vi "AddDesignPatterns.vi"(0 "ClassWriterNative":refnum<class "ClassWriterNative.lvclass">, 1 "ClassItemRefIn":refnum<vi>, 2 "DesignPatterns":string[](array[string]), 5 "error in (no error)":errorcluster) -> (14 "ClassWriterNative":refnum<class "ClassWriterNative.lvclass">, 15 "ClassItemRefOut":refnum<vi>, 17 "Cancelled":bool, 19 "error out":errorcluster)   [LabVIEW 2020, in "ClassWriterNative.lvclass"]
uses:
  ClassWriterNative.lvclass
  Provider_BaseClassInterface/DesignPatternsData.ctl
  Common/LvClass_class/GDSLvClass_PlugIn.ctl
  Common/LvClass_class/GDSLvClass_PlugInTypes.ctl
  Provider_BaseClassInterface/BaseProvider_SubVIs/BaseProvider_DesignPatternsActions.ctl
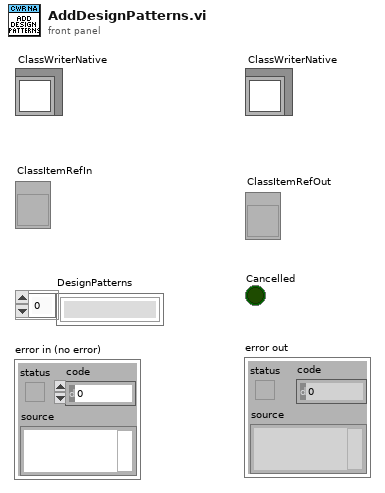
[diagram p1: front panel]
types:
  T1 = typedef "DesignPatternsData.ctl" = cluster{"Type":string, "Patterns":cluster{"ID":string, "Path":path, "Name":string, "Desc":string, "Version":string, "DependenciesID":string[], "OnlyOne":bool}[]}
  T2 = cluster{"Cancel":bool, "ClassProviderName":string, "ClassTemplateUsed":string, "DesignPatterns":T1[], "DataOut":variant, "PlugInVI":path, "DesignPatternID":string, "DesignPatternType":string, "PlugInIDs":string[], "DesignPatternVer":string, "DPIDs":string[], "DpToAdd":cluster{"ID":string, "Path":path, "Name":string, "Desc":string, "Version":string, "DependenciesID":string[], "OnlyOne":bool}[]}
  T3 = cluster{"ID":string, "Path":path, "Name":string, "Desc":string, "Version":string, "DependenciesID":string[], "OnlyOne":bool}[]
  T4 = typedef "GDSLvClass_PlugIn.ctl" = cluster{"Type":T5, "ID":string, "Version":string, "Path":path, "Name":string, "Data":variant}
  T5 = typedef "GDSLvClass_PlugInTypes.ctl" = enum16{"DesignPattern", "MethodTypes"}
  T6 = typedef "BaseProvider_DesignPatternsActions.ctl" = enum16{"AddPatternDialog", "GeneratePattern", "RemovePattern", "CreatePatternMethod", "UpdatePattern"}
  T7 = typedef "GDSLvCLass_ClassSettingsType.ctl" = cluster{"ClassProviderName":string, "ClassTemplateUsed":string, "ClassTemplateVersion":string, "ClassDescription":string, "PlugIns":T4[], "ConnectorPanePattern":string}
  T8 = cluster{"ID":string, "Path":path, "Name":string, "Desc":string, "Version":string, "DependenciesID":string[], "OnlyOne":bool}
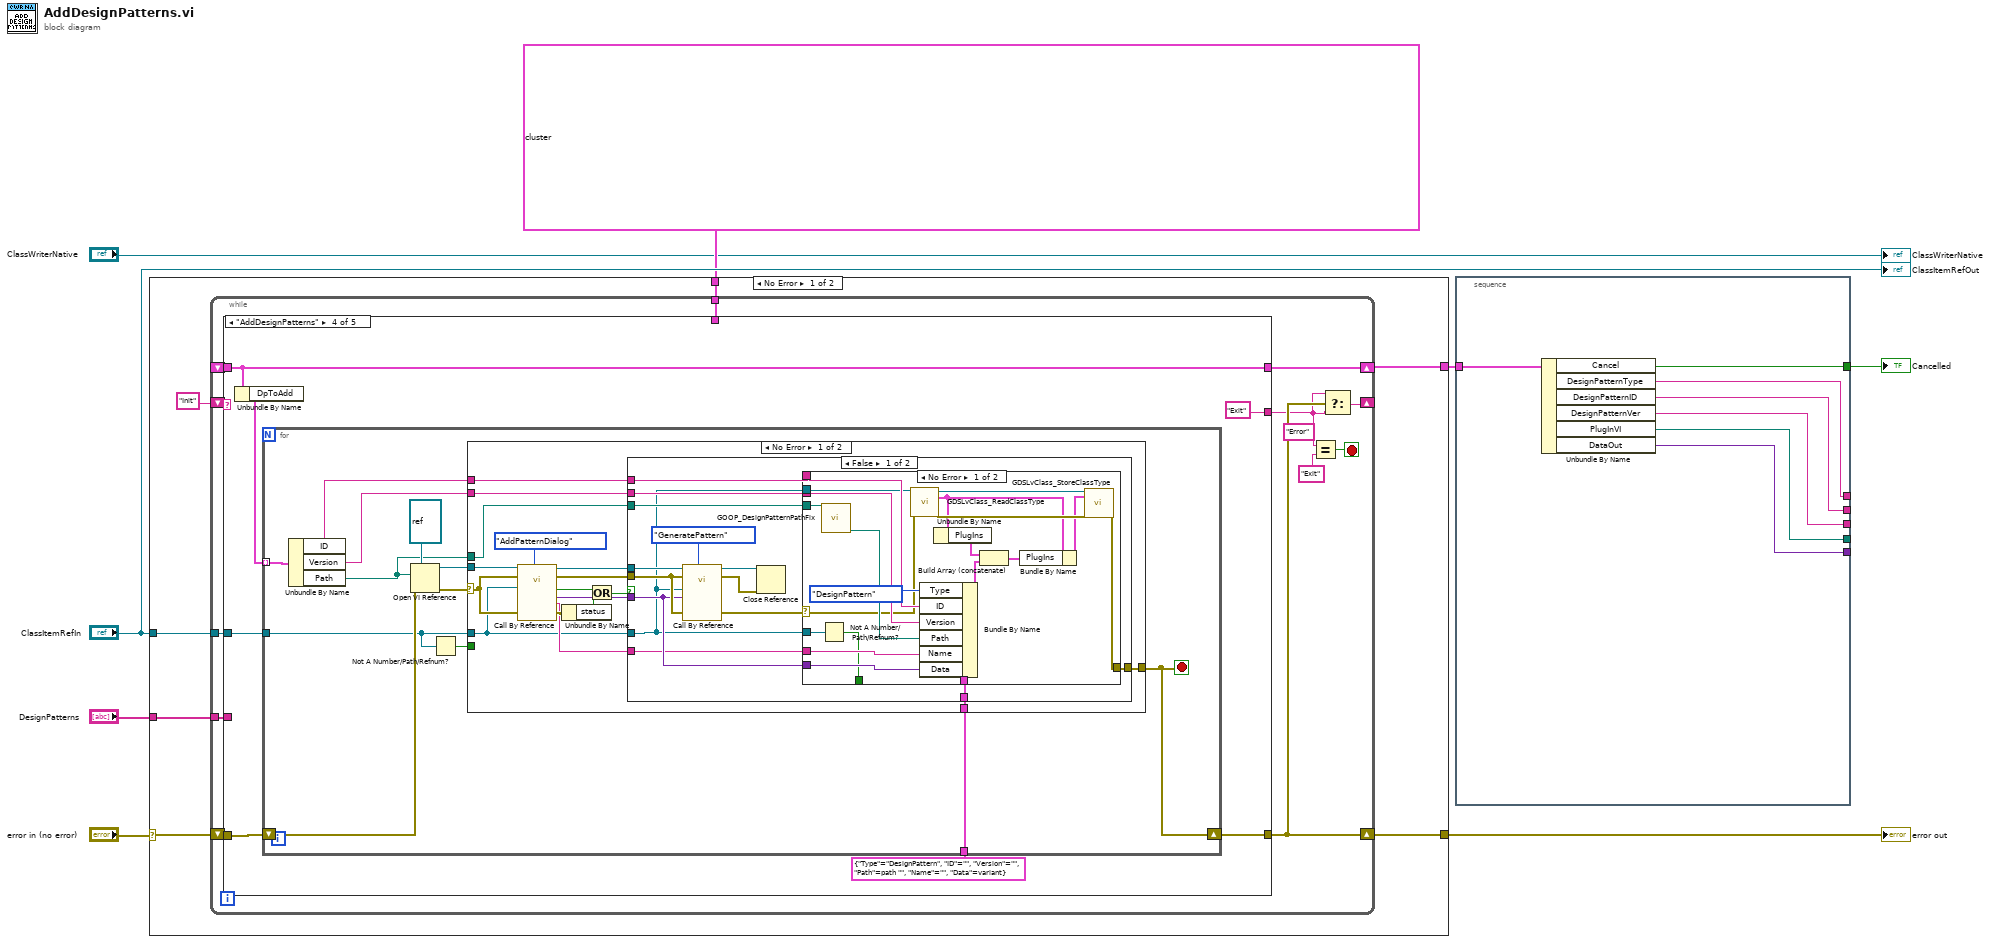
[diagram p0: block diagram]
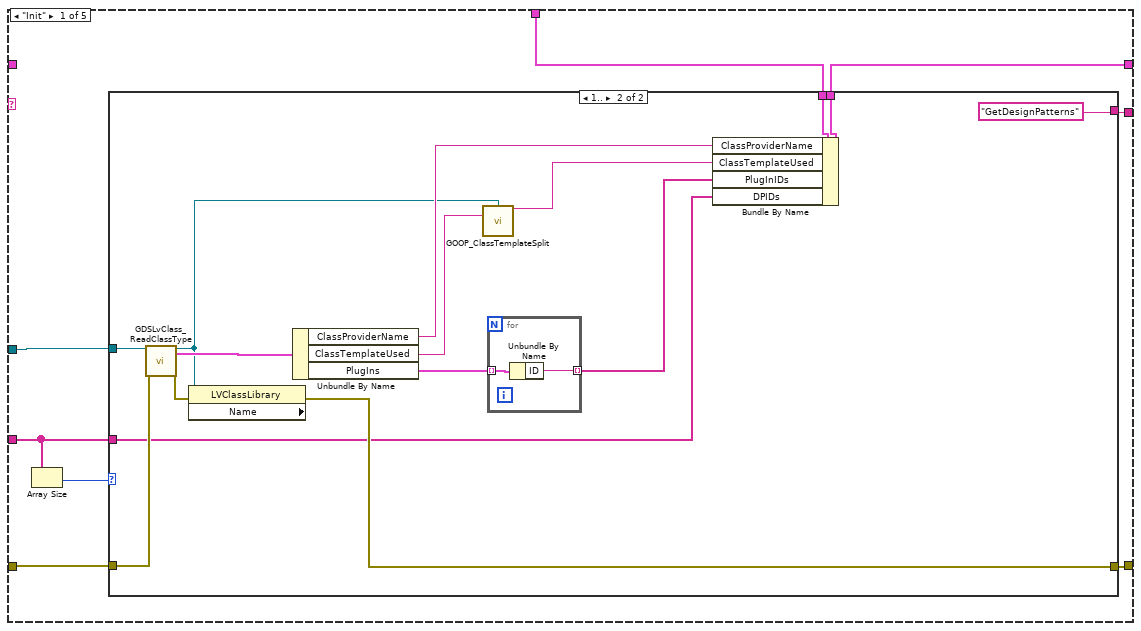
[diagram p2: hidden frame]
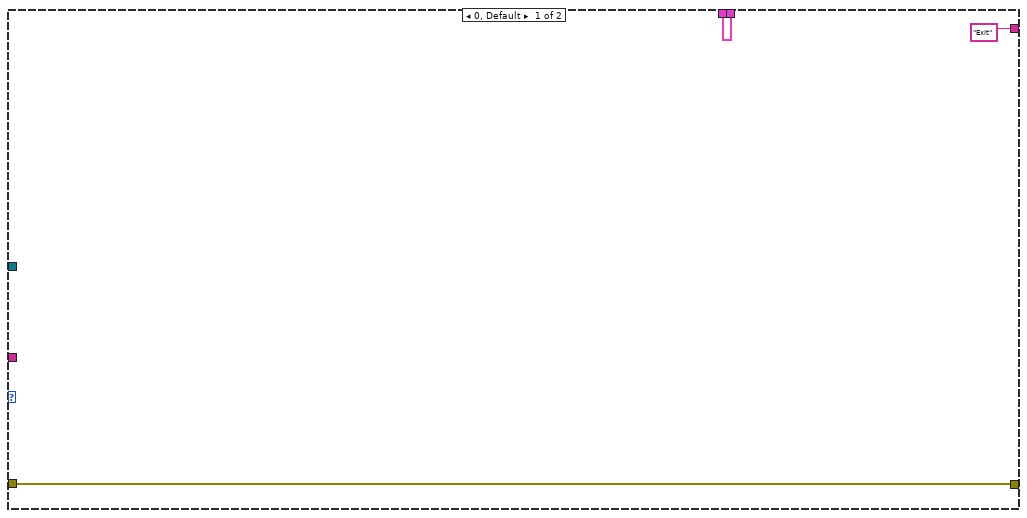
[diagram p3: hidden frame]
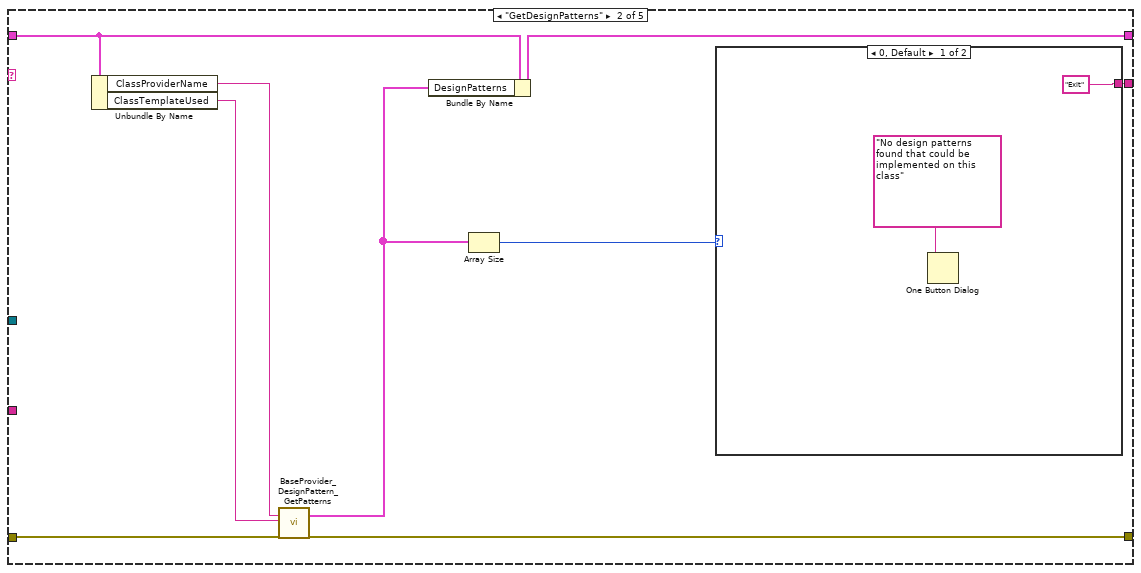
[diagram p4: hidden frame]
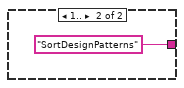
[diagram p5: hidden frame]
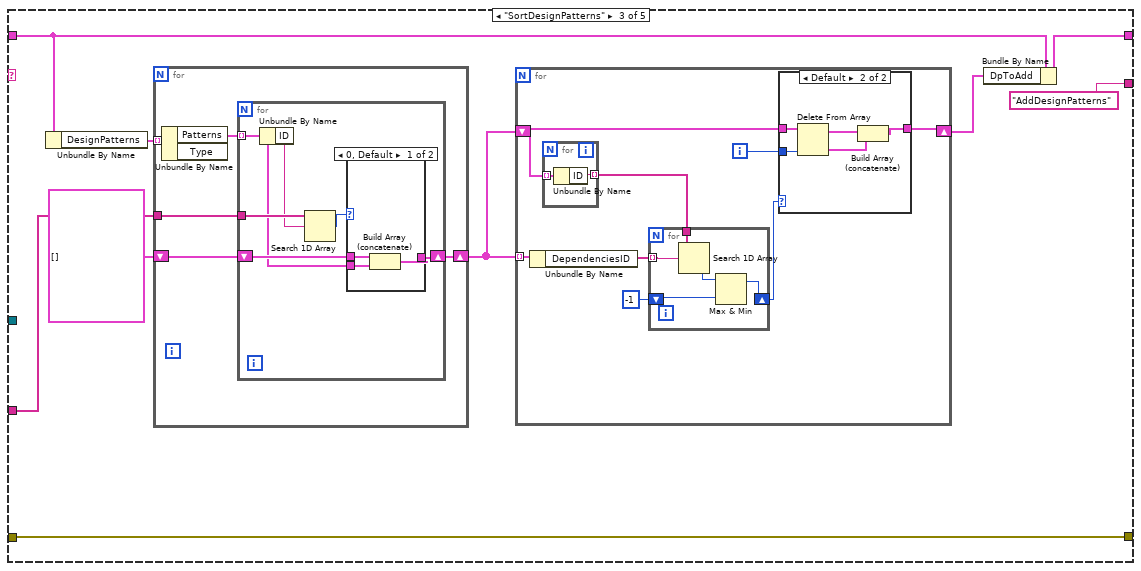
[diagram p6: hidden frame]
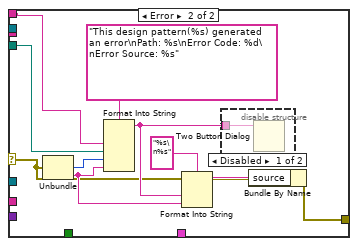
[diagram p9: hidden frame]
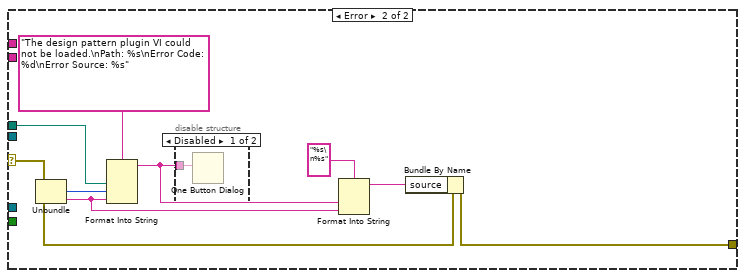
[diagram p12: hidden frame]
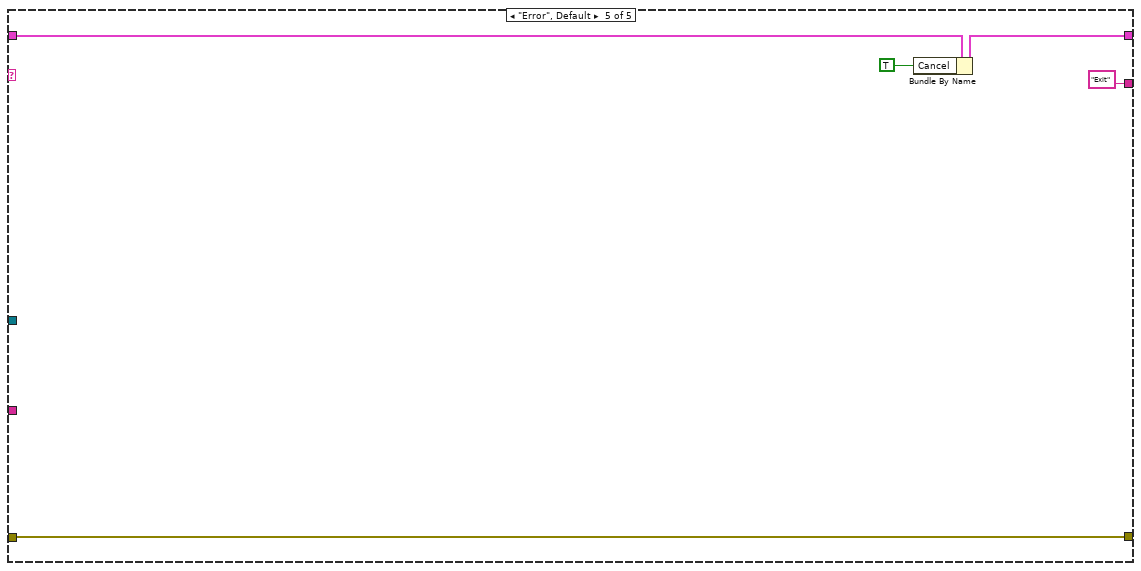
[diagram p14: hidden frame]
diagram:
  n1 = case shown="No Error" "error in (no error)" {
    selector: "error in (no error)" -> [w9 w211]
    tunnel: [w15 w211] -> w5
    tunnel: T2 {"Cancel"=FALSE, "ClassProviderName"="", "ClassTemplateUsed"="", "DesignPatterns"=[], "DataOut"=variant, "PlugInVI"=path "", "DesignPatternID"="", "DesignPatternType"="", "PlugInIDs"=[], "DesignPatternVer"="", "DPIDs"=[], "DpToAdd"=[]} ("output cluster") -> [w13 _]
    tunnel: "ClassItemRefIn" -> [w12 _]
    tunnel: [w11 _] -> w7
    tunnel: "DesignPatterns" -> [w10 _]
    frame No Error {
      n2 = while {
        shift-right: [w22] -> w15
        shift-left: w9 -> [w28]
        shift-right: [w21] -> _
        shift-left: "Init" -> [w25]
        shift-right: [w26] -> w11
        shift-left: _ -> [w27]
        tunnel: w13 -> [w18]
        tunnel: w12 -> [w17]
        tunnel: w10 -> [w16]
        stop <- w23 stop-if-true
        n3 = case shown="\"AddDesignPatterns\"" w25 {
          tunnel: w27 -> [_ w58 w72 w117 w208]
          tunnel: [w31 w57 w71 w117 w207] -> w26
          tunnel: w28 -> [w34 w63 w75 w119 w209]
          tunnel: [w33 w60 w75 w115 w209] -> w22
          tunnel: [w36 w65 "AddDesignPatterns" "Exit" "Exit"] -> w20
          tunnel: w18 -> [w32 _ _ _ _]
          tunnel: w17 -> [w35 _ _ w118 _]
          tunnel: w16 -> [w30 _ w74 _ _]
          frame "Init" {
            n4 = Array Size(array=w30) -> (size(s)=w29:i32)
            n5 = case shown="1.." w29 {
              tunnel: ["Exit" "GetDesignPatterns"] -> w36
              tunnel: w35 -> [_ w53]
              tunnel: w34 -> [w37 w52]
              tunnel: [w37 w49] -> w33
              tunnel: w32 -> [w39 w47]
              tunnel: [w39 w46] -> w31
              tunnel: w30 -> [_ w43]
              frame 0, Default {
              }
              frame 1.. {
                n6 = call "GDSLvClass_ReadClassType.vi"("Class Refnum In"=w53, "error in (no error)"=w52) -> ("Class Refnum Out"=w40:refnum<vi>, "ClassSettings"=w51:T7, "error out"=w50:errorcluster)  [unwired: 15 in]
                n7 = property class="LVClassLibrary" props=["Name"](reference=w40, error in=w50) -> (error out=w49:errorcluster)  [unwired: 2 out]
                n8 = Unbundle By Name(w51) -> ("ClassProviderName"=w48:string, "ClassTemplateUsed"=w42:string, "PlugIns"=w45:T4[])
                n9 = call "GOOP_ClassTemplateSplit.vi"("ClassItemRefIn"=w40, "FullClassTemplate"=w42) -> ("StandardTemplate"=w41:string)  [unwired: 12 in, 1 out]
                n10 = for {
                  tunnel: w45 -> [w56] mode=indexing
                  tunnel: [w55] -> w44 mode=indexing
                  n11 = Unbundle By Name(w56) -> ("ID"=w55:string)
                }
                n12 = Bundle By Name(cluster=w47, "ClassProviderName"=w48, "ClassTemplateUsed"=w41, "PlugInIDs"=w44, "DPIDs"=w43) -> (w46:T2)
              }
            }
          }
          frame "GetDesignPatterns" {
            n13 = Unbundle By Name(w58) -> ("ClassProviderName"=w62:string, "ClassTemplateUsed"=w61:string)
            n14 = call "BaseProvider_DesignPattern_GetPatterns.vi"("FilterOnProviders(Ignored If Empty)"=w62, "FilterOnTemplate(Ignored If Empty)"=w61, "error in (no error)"=w63) -> ("DesignPatterns"=w59:T1[], "error out"=w60:errorcluster)  [unwired: 15 in]
            n15 = Bundle By Name(cluster=w58, "DesignPatterns"=w59) -> (w57:T2)
            n16 = Array Size(array=w59) -> (size(s)=w64:i32)
            n17 = case shown="0, Default" w64 {
              tunnel: ["Exit" "SortDesignPatterns"] -> w65
              frame 0, Default {
                n18 = One Button Dialog(message="No design patterns found that could be implemented on this class" ("format string")) -> ()  [unwired: 1 in, 1 out]
              }
              frame 1.. {
              }
            }
          }
          frame "SortDesignPatterns" {
            n19 = Unbundle By Name(w72) -> ("DesignPatterns"=w76:T1[])
            n20 = for {
              tunnel: w76 -> [w103] mode=indexing
              tunnel: w74 -> [w101]
              shift-right: [w99] -> w73
              shift-left: T3 [] -> [w100]
              n21 = Unbundle By Name(w103) -> ("Patterns"=w102:T3)  [unwired: 1 out]
              n22 = for {
                tunnel: w102 -> [w104] mode=indexing
                tunnel: w101 -> [w109]
                shift-right: [w105] -> w99
                shift-left: w100 -> [w106]
                n23 = Unbundle By Name(w104) -> ("ID"=w108:string)
                n24 = Search 1D Array(1D array=w109, element=w108) -> (index of element=w107:i32)  [unwired: 1 in]
                n25 = case shown="0, Default" w107 {
                  tunnel: w106 -> [w112 w113]
                  tunnel: [w111 w113] -> w105
                  tunnel: w104 -> [w110 _]
                  frame 0, Default {
                    n26 = Build Array (concatenate)(w112, w110) -> (w111:T3)
                  }
                  frame -1 {
                  }
                }
              }
            }
            n27 = for {
              tunnel: w73 -> [w85] mode=indexing
              shift-right: [w79] -> w70
              shift-left: w73 -> [w81]
              i -> [w78]
              n28 = Unbundle By Name(w85) -> ("DependenciesID"=w84:string[])
              n29 = for {
                tunnel: w81 -> [w98] mode=indexing
                tunnel: [w97] -> w83 mode=indexing
                n30 = Unbundle By Name(w98) -> ("ID"=w97:string)
              }
              n31 = for {
                tunnel: w84 -> [w96] mode=indexing
                tunnel: w83 -> [w95]
                shift-right: [w92] -> w80
                shift-left: -1 -> [w93]
                n32 = Search 1D Array(1D array=w95, element=w96) -> (index of element=w94:i32)  [unwired: 1 in]
                n33 = Max & Min(x=w94, y=w93) -> (max(x,y)=w92:i32)  [unwired: 1 out]
              }
              n34 = case shown="Default" w80 {
                tunnel: w81 -> [w86 w91]
                tunnel: [w86 w87] -> w79
                tunnel: w78 -> [_ w90]
                frame -1 {
                }
                frame Default {
                  n35 = Delete From Array(array=w91, index=w90) -> (deleted portion=w88:T8, array with subset deleted=w89:T3)  [unwired: 1 in]
                  n36 = Build Array (concatenate)(w89, w88) -> (w87:T3)
                }
              }
            }
            n37 = Bundle By Name(cluster=w72, "DpToAdd"=w70) -> (w71:T2)
          }
          frame "AddDesignPatterns" {
            n38 = Unbundle By Name(w117) -> ("DpToAdd"=w120:T3)
            n39 = for {
              tunnel: w120 -> [w128] mode=indexing
              shift-right: [w121] -> w115
              shift-left: w119 -> [w127]
              tunnel: w118 -> [w123]
              tunnel: T4 {"Type"=enum."DesignPattern", "ID"="", "Version"="", "Path"=path "", "Name"="", "Data"=variant} ("PlugIn") -> [w126]
              stop <- w121 stop-if-true
              n40 = Unbundle By Name(w128) -> ("ID"=w125:string, "Version"=w124:string, "Path"=w129:path)
              n41 = Open VI Reference(type specifier VI Refnum (for type only)=refnum<vi> refnum, vi path=w129, error in (no error)=w127) -> (vi reference=w131:refnum<vi>, error out=w130:errorcluster)  [unwired: 3 in]
              n42 = Not A Number/Path/Refnum?(number/path/refnum=w123) -> (NaN/Path/Refnum?=w122:bool)
              n43 = case shown="No Error" w130 {
                selector: w130 -> [w141 w201]
                tunnel: w131 -> [w149 _]
                tunnel: w129 -> [w136 w202]
                tunnel: w123 -> [w134 _]
                tunnel: w126 -> [w139 _]
                tunnel: w125 -> [w138 _]
                tunnel: w124 -> [w137 _]
                tunnel: w122 -> [_ _]
                tunnel: [w133 w196] -> w121
                frame No Error {
                  n44 = call-by-ref "?"(reference=w149, error in=w141, "Action"=BaseProvider_DesignPatternsActions."AddPatternDialog", 8:"error in (no error)"=w141, "ClassRefToActOn"=w134) -> (reference out=w143:refnum<vi>, error out=w142:errorcluster, 0:"error out"=w148:errorcluster, "Name"=w135:string, "DataOut"=w140:variant, "Cancelled"=w147:bool)  [unwired: 5 in]
                  n45 = Unbundle By Name(w148) -> ("status"=w145:bool)
                  n46 = Or(x=w147, y=w145) -> (x .or. y?=w144:bool)
                  n47 = case shown="False" w144 {
                    tunnel: w143 -> [w163 _]
                    tunnel: w134 -> [w151 _]
                    tunnel: w142 -> [w161 w195]
                    tunnel: w140 -> [w156 _]
                    tunnel: w139 -> [w157 _]
                    tunnel: w138 -> [w155 _]
                    tunnel: w137 -> [w154 _]
                    tunnel: w136 -> [w153 _]
                    tunnel: w135 -> [w152 _]
                    tunnel: [w150 w195] -> w133
                    frame False {
                      n48 = call-by-ref "?"(reference=w163, error in=w161, "Action"=BaseProvider_DesignPatternsActions."GeneratePattern", 8:"error in (no error)"=w161, "DataIn"=w156, "ClassRefToActOn"=w151) -> (reference out=w160:refnum<vi>, error out=w159:errorcluster, 0:"error out"=w158:errorcluster)  [unwired: 4 in, 3 out]
                      n49 = Close Reference(reference=w160, error in (no error)=w159) -> ()  [unwired: 1 out]
                      n50 = case shown="No Error" w158 {
                        selector: w158 -> [w164 w185]
                        tunnel: w157 -> [w175 _]
                        tunnel: w156 -> [w174 _]
                        tunnel: w155 -> [w173 w191]
                        tunnel: w154 -> [w172 _]
                        tunnel: w153 -> [w167 w190]
                        tunnel: w151 -> [w171 _]
                        tunnel: w152 -> [w170 _]
                        tunnel: w151 -> [w169 _]
                        tunnel: [w168 _] -> _
                        tunnel: [w165 w184] -> w150
                        frame No Error {
                          n51 = Not A Number/Path/Refnum?(number/path/refnum=w169) -> (NaN/Path/Refnum?=w168:bool)
                          n52 = call "GOOP_DesignPatternPathFix.vi"("ViPathIn"=w167) -> ("RelativeVIPathOut(ToStoreInLvClass)"=w166:path)  [unwired: 6 in, 4 out]
                          n53 = call "GDSLvClass_ReadClassType.vi"("Class Refnum In"=w171, "error in (no error)"=w164) -> ("Class Refnum Out"=w183:refnum<vi>, "ClassSettings"=w180:T7, "error out"=w182:errorcluster)  [unwired: 15 in]
                          n54 = Bundle By Name(cluster=w175, "Type"=GDSLvClass_PlugInTypes."DesignPattern", "ID"=w173, "Version"=w172, "Path"=w166, "Name"=w170, "Data"=w174) -> (w177:T4)
                          n55 = Unbundle By Name(w180) -> ("PlugIns"=w179:T4[])
                          n56 = Build Array (concatenate)(w179, w177) -> (w178:T4[])
                          n57 = Bundle By Name(cluster=w180, "PlugIns"=w178) -> (w181:T7)
                          n58 = call "GDSLvClass_StoreClassType.vi"("Class Refnum In"=w183, "ClassSettings"=w181, "error in (no error)"=w182) -> ("error out"=w165:errorcluster)  [unwired: 15 in, 1 out]
                        }
                        frame Error {
                          n59 = Unbundle(w185) -> ("code"=w192:i32, "source"=w186:string)  [unwired: 1 out]
                          n60 = Format Into String(format string="This design pattern(%s) generated an error\nPath: %s\nError Code: %d\nError Source: %s" ("message"), w191, w190, w192, w186) -> (resulting string=w187:string)  [unwired: 2 in, 1 out]
                          n61 = Format Into String(format string="%s\n%s", w187, w186) -> (resulting string=w188:string)  [unwired: 2 in, 1 out]
                          n62 = disable-structure shown="Disabled" {
                            disable-tunnel: w187 -> [w194 _]
                            frame Disabled {
                              n63 = Two Button Dialog(message=w194) -> ()  [unwired: 2 in, 1 out]
                            }
                            frame Enabled {
                            }
                          }
                          n64 = Bundle By Name(cluster=w185, "source"=w188) -> (w184:errorcluster)
                        }
                      }
                    }
                    frame True {
                    }
                  }
                }
                frame Error {
                  n65 = Unbundle(w201) -> ("code"=w203:i32, "source"=w198:string)  [unwired: 1 out]
                  n66 = Format Into String(format string="The design pattern plugin VI could not be loaded.\nPath: %s\nError Code: %d\nError Source: %s" ("message"), w202, w203, w198) -> (resulting string=w199:string)  [unwired: 2 in, 1 out]
                  n67 = disable-structure shown="Disabled" {
                    disable-tunnel: w199 -> [w205 _]
                    frame Disabled {
                      n68 = One Button Dialog(message=w205) -> ()  [unwired: 1 in, 1 out]
                    }
                    frame Enabled {
                    }
                  }
                  n69 = Format Into String(format string="%s\n%s", w199, w198) -> (resulting string=w197:string)  [unwired: 2 in, 1 out]
                  n70 = Bundle By Name(cluster=w201, "source"=w197) -> (w196:errorcluster)
                }
              }
            }
          }
          frame "Error", Default {
            n71 = Bundle By Name(cluster=w208, "Cancel"=TRUE) -> (w207:T2)
          }
        }
        n72 = Equal?(x=w20, y="Exit") -> (x = y?=w23:bool)
        n73 = Select(t="Error", s=w22, f=w20) -> (s? t:f=w21:string)
      }
    }
    frame Error {
    }
  }
  "error out" <- w5
  n74 = stacked-sequence {
    tunnel: w7 -> [w218]
    tunnel: [w217] -> w6
    tunnel: [w216] -> _
    tunnel: [w215] -> _
    tunnel: [w214] -> _
    tunnel: [w213] -> _
    tunnel: [w212] -> _
    frame #0 {
      n75 = Unbundle By Name(w218) -> ("Cancel"=w217:bool, "DesignPatternType"=w213:string, "DesignPatternID"=w214:string, "DesignPatternVer"=w212:string, "PlugInVI"=w216:path, "DataOut"=w215:variant)
    }
  }
  "Cancelled" <- w6
  "ClassWriterNative" <- "ClassWriterNative"
  "ClassItemRefOut" <- "ClassItemRefIn"
